vi "constant_jdp_sqlite.vi"() -> (0 "jdp_sqlite_mapper":refnum<class "Mapper.lvclass">, 1 "jdp_sqlite_dbc":refnum<class "DBC.lvclass">)   [LabVIEW 2020, in "ORM_API_jdp.lvlib"]
uses:
  ORM_API_jdp.lvlib
  <vilib>/Viviota/shared/ORM_sqlite_jdp.lvlibp/dbc/DBC.lvclass
  <vilib>/Viviota/shared/ORM_sqlite_jdp.lvlibp/PGJDPMapper/Mapper.lvclass
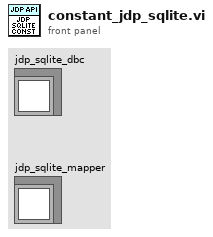
[diagram p1: front panel]
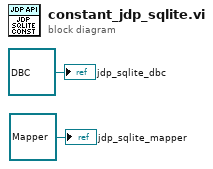
[diagram p0: block diagram]
diagram:
  "jdp_sqlite_dbc" <- refnum<class "DBC.lvclass"> refnum ("ORM_sqlite_jdp.lvlibp:DBC.lvclass")
  "jdp_sqlite_mapper" <- refnum<class "Mapper.lvclass"> refnum ("ORM_sqlite_jdp.lvlibp:Mapper.lvclass")
